vi "Prueba Motor.vi"() -> ()   [LabVIEW 2021]
uses:
  <vilib>/DAQmx/read.llb/DAQmx Read (Counter DBL 1Chan 1Samp).vi
  <vilib>/DAQmx/write.llb/DAQmx Write (Analog DBL 1Chan 1Samp).vi
  <vilib>/DAQmx/write.llb/DAQmx Write (Digital 1D Bool 1Chan 1Samp).vi
  <vilib>/DAQmx/create/channels.llb/DAQmx Create Channel (CI-Position-Angular Encoder).vi
  <vilib>/DAQmx/create/channels.llb/DAQmx Create Channel (AO-Voltage-Basic).vi
  <vilib>/DAQmx/create/channels.llb/DAQmx Create Channel (DO-Digital Output).vi
  <vilib>/DAQmx/miscellaneous.llb/DAQmx Fill In Error Info.vi
  <vilib>/Utility/file.llb/Write Delimited Spreadsheet (DBL).vi
  <resource>/objmgr/daqmx.rc
panel:
  out "error out":errorcluster
  in  "stop":bool
  out "Ángulo [°]":dbl(graph)
  in  "Archivo":path=path "C:/Users/labfisica/Documents/GitHub/Codigo_Proyecto_Pendulo/Logs/Prueba motores.txt"
  in  "Motor 2":bool
  in  "Motor 1":bool
  in  "AO [V]":dbl(slide) scale=0.0..5.0
  in  "lines":tag="Dev1/port0/line2, Dev1/port0/line1"
  in  "counter":tag="Dev1/ctr0"
  in  "physical channels":tag="Dev1/ao0"
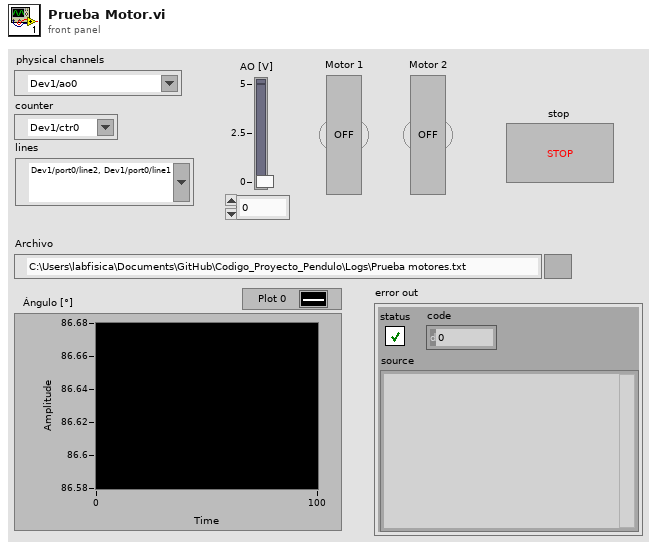
[diagram p1: front panel]
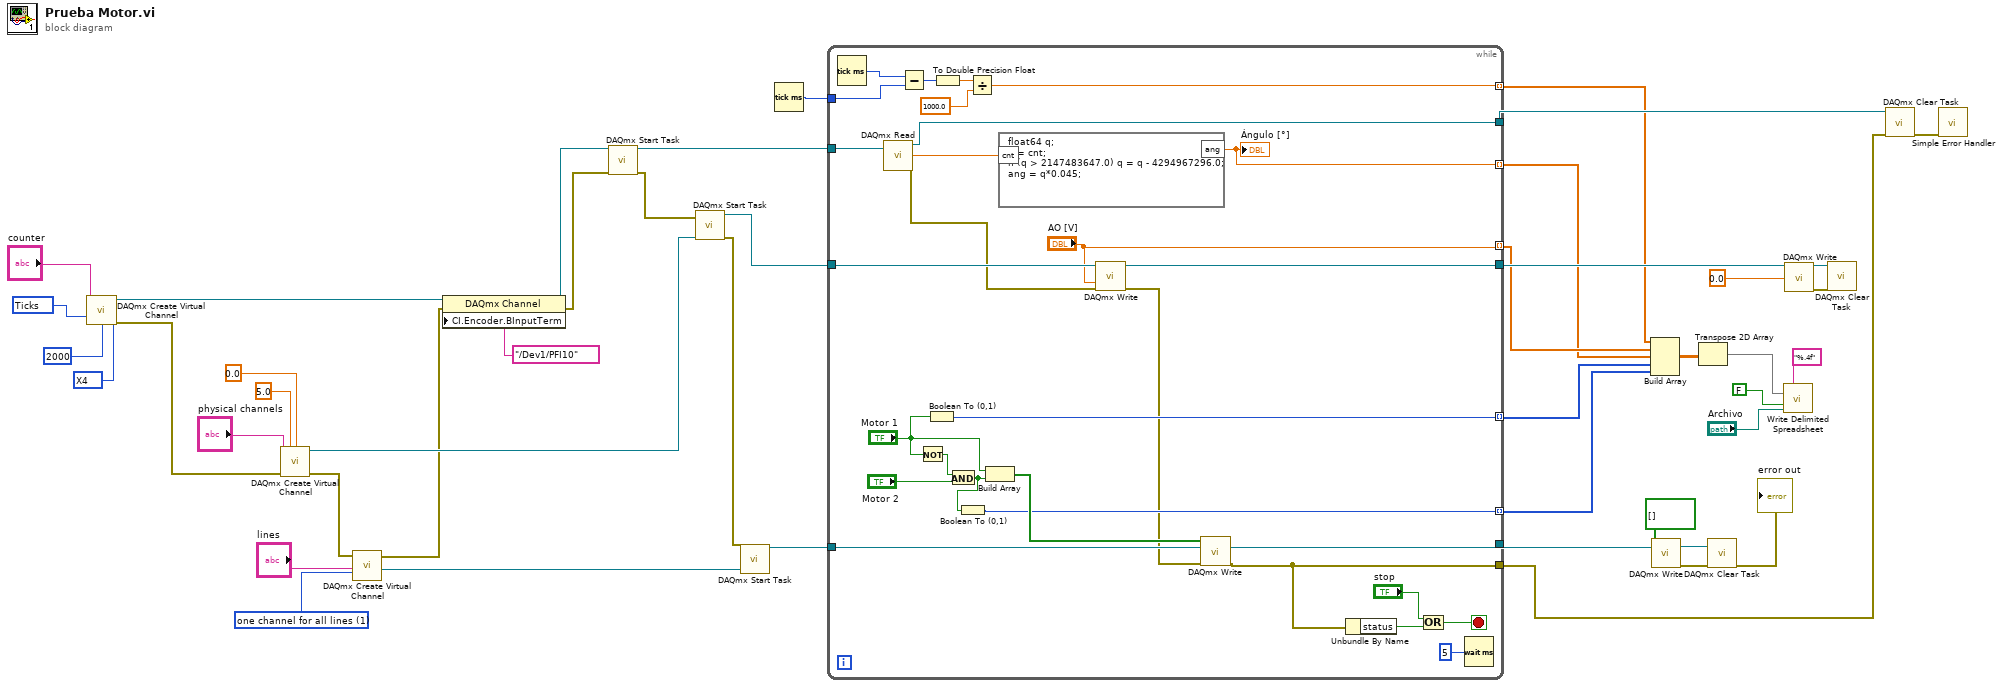
[diagram p0: block diagram]
diagram:
  w38 = 1 items=["one channel for each line", "one channel for all lines"] ("line grouping")
  w35 = 10304 items=["Degrees"=10146, "Radians"=10273, "Ticks"=10304, "From Custom Scale"=10065] ("units")
  w45 = 10092 items=["X1"=10090, "X2"=10091, "X4"=10092, "Two Pulse Counting"=10313] ("decoding type")
  n1 = call-poly <vilib>:"DAQmx Create Virtual Channel.vi"("counter"="counter", "decoding type"=w45, "units"=w35, "pulses per revolution"=u32 2000) -> ("task out"=w33:refnum<k21>, "error out"=w31:errorcluster)  [unwired: 10 in]
  n2 = call-poly <vilib>:"DAQmx Create Virtual Channel.vi"("maximum value"=5.0, "minimum value"=0.0, "physical channels"="physical channels", "error in"=w31) -> ("task out"=w37:refnum<k21>, "error out"=w30:errorcluster)  [unwired: 10 in]
  n3 = call-poly <vilib>:"DAQmx Create Virtual Channel.vi"("lines"="lines", "line grouping"=w38, "error in"=w30) -> ("task out"=w36:refnum<k21>, "error out"=w29:errorcluster)  [unwired: 11 in]
  n4 = property class="DAQmx Channel"(reference=w33, error in=w29, "CI.Encoder.BInputTerm"=tag "/Dev1/PFI10") -> (reference out=w26:refnum<k21>, error out=w32:errorcluster)
  n5 = call <vilib>:"DAQmx Start Task.vi"("task/channels in"=w26, "error in"=w32) -> ("task out"=w25:refnum<k21>, "error out"=w28:errorcluster)  [unwired: 12 in]
  n6 = call <vilib>:"DAQmx Start Task.vi"("task/channels in"=w37, "error in"=w28) -> ("task out"=w23:refnum<k21>, "error out"=w27:errorcluster)  [unwired: 12 in]
  n7 = call <vilib>:"DAQmx Start Task.vi"("task/channels in"=w36, "error in"=w27) -> ("task out"=w22:refnum<k21>)  [unwired: 12 in, 1 out]
  n8 = Tick Count (ms)() -> (millisecond timer value=w24:u32)
  n9 = while {
    tunnel: w25 -> [w74]
    tunnel: w24 -> [w70]
    tunnel: w23 -> [w68]
    tunnel: w22 -> [w65]
    tunnel: [w63] -> w9 mode=indexing
    tunnel: [w62] -> w8 mode=indexing
    tunnel: [w60] -> w12 mode=indexing
    tunnel: [w59] -> w10 mode=indexing
    tunnel: [w56] -> w15
    tunnel: [w53] -> w16
    tunnel: [w58] -> w14
    tunnel: [w50] -> w2
    tunnel: ["AO [V]"] -> w11 mode=indexing
    stop <- w49 stop-if-true
    n10 = Tick Count (ms)() -> (millisecond timer value=w69:u32)
    n11 = call-poly <vilib>:"DAQmx Read.vi"("task/channels in"=w74) -> ("task out"=w53:refnum<k21>, "data"=w46:dbl, "error out"=w57:errorcluster)  [unwired: 12 in]
    n12 = Subtract(x=w69, y=w70) -> (x-y=w72:u32)
    n13 = Not(x="Motor 1") -> (.not. x?=w67:bool)
    n14 = Boolean To (0,1)(Boolean="Motor 1") -> (0, 1=w63:i16)
    n15 = To Double Precision Float(number=w72) -> (double precision float=w73:dbl)
    n16 = And(x=w67, y="Motor 2") -> (x .and. y?=w51:bool)
    n17 = Boolean To (0,1)(Boolean=w51) -> (0, 1=w62:i16)
    n18 = Divide(x=w73, y=1000.0) -> (x/y=w60:dbl)
    n19 = Build Array("Motor 1", w51) -> (w66:bool[])
    n20 = formula code="float64 q;\nq = cnt;\nif (q > 2147483647.0) q = q - 4294967296.0;\nang = q*0.045;"("cnt"=w46) -> ("ang"=w59:dbl)
    "Ángulo [°]" <- w59
    n21 = call-poly <vilib>:"DAQmx Write.vi"("task/channels in"=w68, "data"="AO [V]", "error in"=w57) -> ("task out"=w56:refnum<k21>, "error out"=w55:errorcluster)  [unwired: 10 in, 1 out]
    n22 = call-poly <vilib>:"DAQmx Write.vi"("task/channels in"=w65, "data"=w66, "error in"=w55) -> ("task out"=w58:refnum<k21>, "error out"=w50:errorcluster)  [unwired: 10 in, 1 out]
    n23 = Unbundle By Name(w50) -> ("status"=w47:bool)
    n24 = Or(x="stop", y=w47) -> (x .or. y?=w49:bool)
    n25 = Wait (ms)(milliseconds to wait=u32 5) -> ()  [unwired: 1 out]
  }
  n26 = Build Array(w12, w11, w10, w9, w8) -> (w7:dbl[][])
  n27 = call-poly <vilib>:"DAQmx Write.vi"("task/channels in"=w14, "data"=bool[] []) -> ("task out"=w19:refnum<k21>, "error out"=→"error out":errorcluster)  [unwired: 11 in, 1 out]
  n28 = Transpose 2D Array(2D array=w7) -> (transposed array=w6:dbl[][])
  n29 = call <vilib>:"DAQmx Clear Task.vi"("task in"=w19) -> ()  [unwired: 14 in, 1 out]
  n30 = call-poly <vilib>:"Write Delimited Spreadsheet.vi"("file path (dialog if empty)"="Archivo", "format (%.3f)"="%.4f", "2D data"=w6, "append to file? (new file:F)"=FALSE) -> ()  [unwired: 10 in, 2 out]
  n31 = call-poly <vilib>:"DAQmx Write.vi"("task/channels in"=w15, "data"=0.0) -> ("task out"=w1:refnum<k21>, "error out"=w13:errorcluster)  [unwired: 11 in, 1 out]
  n32 = call <vilib>:"DAQmx Clear Task.vi"("task in"=w1, "error in"=w13) -> ()  [unwired: 13 in, 1 out]
  n33 = call <vilib>:"DAQmx Clear Task.vi"("task in"=w16, "error in"=w2) -> ("error out"=w17:errorcluster)  [unwired: 13 in]
  n34 = call <vilib>:"Simple Error Handler.vi"("error in (no error)"=w17) -> ()  [unwired: 4 in, 5 out]
